vi "Create Class.vi"(8 "error in (no error)":errorcluster, 11 "Mock Class Generator in":refnum<class "Mock Class Generator.lvclass">) -> (0 "error out":errorcluster, 2 "Created Class":path[](array[path]), 3 "Mock Class Generator out":refnum<class "Mock Class Generator.lvclass">)   [LabVIEW 2020, in "Mock Class Generator.lvclass"]
uses:
  Mock Class Generator.lvclass
  Mock Class Generator.lvclass/Mock Class Generator.ctl
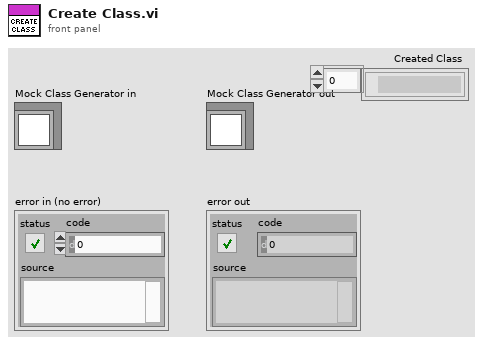
[diagram p1: front panel]
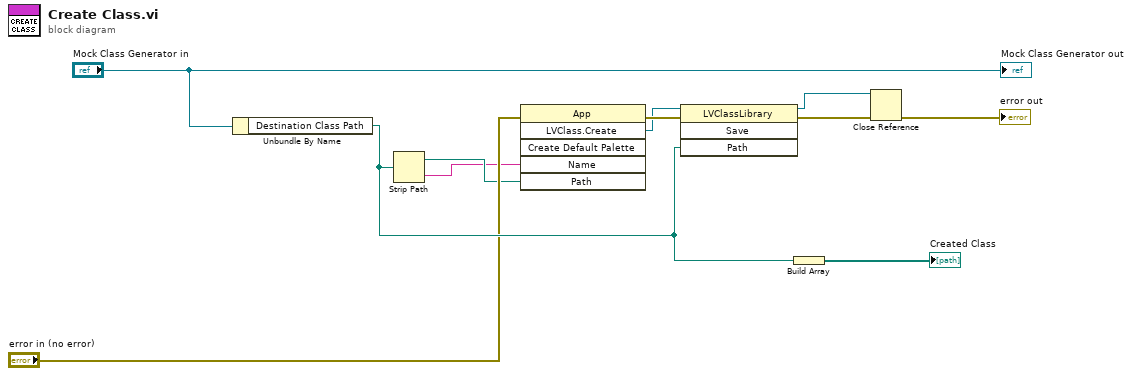
[diagram p0: block diagram]
diagram:
  n1 = Unbundle By Name("Mock Class Generator in") -> ("Destination Class Path"=w8:path)
  n2 = Strip Path(path=w8) -> (stripped path=w5:path, name=w4:string)
  n3 = invoke class="App" method="LVClass.Create"(error in="error in (no error)", "Name"=w4, "Path"=w5) -> (error out=w3:errorcluster, "LVClass.Create"=w2:refnum<vi>)  [unwired: 3 in, 4 out]
  n4 = invoke class="LVClassLibrary" method="Save"(reference=w2, error in=w3, "Path"=w8) -> (reference out=w10:refnum<vi>, error out=w7:errorcluster)  [unwired: 1 in, 2 out]
  n5 = Build Array(w8) -> (→"Created Class":path[])
  n6 = Close Reference(reference=w10, error in (no error)=w7) -> (error out=→"error out":errorcluster)
  "Mock Class Generator out" <- "Mock Class Generator in"
